vi "add_moving_vertical_cursor.vi"(8 "error in":errorcluster, 10 "Cursor Position":dbl, 11 "reference in":refnum<vi>) -> (0 "error out":errorcluster, 3 "reference out":refnum<vi>)   [LabVIEW 2025, in "tSNIP.lvlib"]
uses:
  tSNIP.lvlib
  <vilib>/Utility/miscctls.llb/LVCursorListTypeDef.ctl
panel:
  in  "Name":string="Cursor 0"
  in  "Cursor Color":u32(colorbox)=16711680
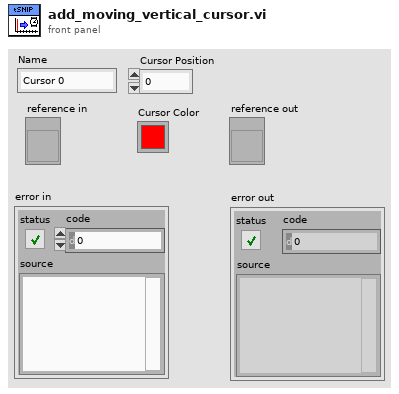
[diagram p1: front panel]
types:
  T1 = typedef "LVCursorListTypeDef.ctl" = cluster{"Name":string, "Color":u32, "Style":u8, "Point Style":u8, "Name Visible":bool, "Allow Drag":bool, "Cursor Mode":u32, "Plot":i32, "Index":i32, "Position":cluster{"X":dbl, "Y":dbl}, "X Scale":u32, "Y Scale":u32, "Watch Plots":i32[], "Watch All Plots":bool, "Plot Area":i32, "Label Offset":cluster{"X":dbl, "Y":dbl}}[]
  T2 = cluster{"Name":string, "Color":u32, "Style":u8, "Point Style":u8, "Name Visible":bool, "Allow Drag":bool, "Cursor Mode":u32, "Plot":i32, "Index":i32, "Position":cluster{"X":dbl, "Y":dbl}, "X Scale":u32, "Y Scale":u32, "Watch Plots":i32[], "Watch All Plots":bool, "Plot Area":i32, "Label Offset":cluster{"X":dbl, "Y":dbl}}
  T3 = cluster{"Name":string, "Color":u32, "Style":u8, "Point Style":u8, "Name Visible":bool, "Allow Drag":bool, "Cursor Mode":u32, "Plot":i32, "Index":i32, "Position":cluster{"X":dbl, "Y":dbl}, "X Scale":u32, "Y Scale":u32, "Watch Plots":i32[], "Watch All Plots":bool, "Plot Area":i32, "Label Offset":cluster{"X":dbl, "Y":dbl}}[]
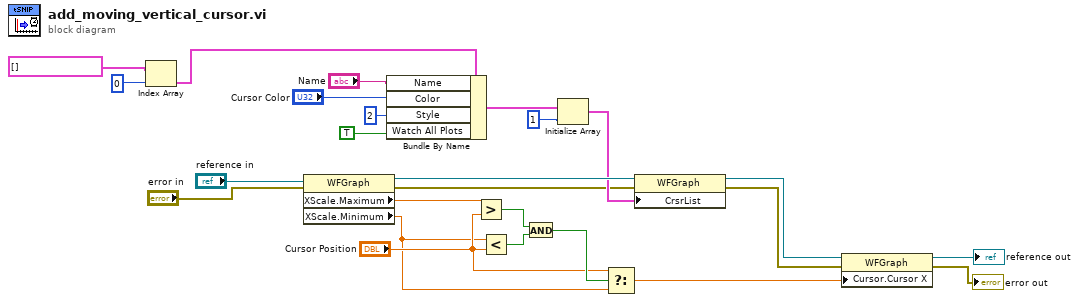
[diagram p0: block diagram]
diagram:
  n1 = Index Array(array=T1 [] ("Cursor List"), index=0) -> (element=w17:T2)
  n2 = property class="WFGraph"(reference="reference in", error in="error in") -> (reference out=w21:refnum<vi>, error out=w1:errorcluster, "XScale.Maximum"=w9:dbl, "XScale.Minimum"=w4:dbl)
  n3 = Bundle By Name(cluster=w17, "Name"="Name", "Color"="Cursor Color", "Style"=u8 2, "Watch All Plots"=TRUE) -> (w12:T2)
  n4 = Greater?(x=w9, y="Cursor Position") -> (0:w8:bool)
  n5 = Less?(x=w4, y="Cursor Position") -> (x < y?=w7:bool)
  n6 = And(x=w8, y=w7) -> (x .and. y?=w6:bool)
  n7 = Initialize Array(w12, 1 ("dimension size")) -> (w10:T3)
  n8 = Select(t="Cursor Position", s=w6, f=w4) -> (s? t:f=w3:dbl)
  n9 = property class="WFGraph"(reference=w21, error in=w1, "CrsrList"=w10) -> (reference out=w20:refnum<vi>, error out=w2:errorcluster)
  n10 = property class="WFGraph"(reference=w20, error in=w2, "Cursor.Cursor X"=w3) -> (reference out=→"reference out":refnum<vi>, error out=→"error out":errorcluster)
